vi "libssh2_channel_read_ex.vi"(8 "error in (no error)":errorcluster, 9 "buffer length":i32=1024, 10 "stream id":i32, 11 "channel":T1) -> (0 "error out":errorcluster, 2 "buffer":u8[](array[numeric]))   [LabVIEW 2017, in "libssh2.lvlib"]
doc: "Read data from a channel.\nAll channel streams have one standard input/output substream (<B>stream id</B> = 0), and may have up to 2^32 extended data streams as identified by the selected <B>stream id</B>. The SSH-2 protocol currently defines a standard stream ID of 1 to be the stderr substream."
uses:
  libssh2.lvlib
  Channel Refnum.ctl
  Acquire Session.vi
  Release Session.vi
  Not A Channel.vi
  <vilib>/Utility/error.llb/Error Cluster From Error Code.vi
  Global Settings.vi
  Read Channel Refnum.vi
  Read Session Refnum.vi
  <vilib>/Utility/semaphor.llb/Acquire Semaphore.vi
  <vilib>/Utility/semaphor.llb/Release Semaphore.vi
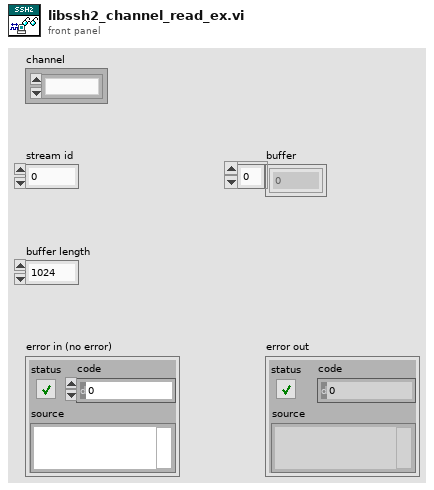
[diagram p1: front panel]
types:
  T1 = typedef "libssh2.lvlib/Channel Refnum.ctl" = refnum<k1>
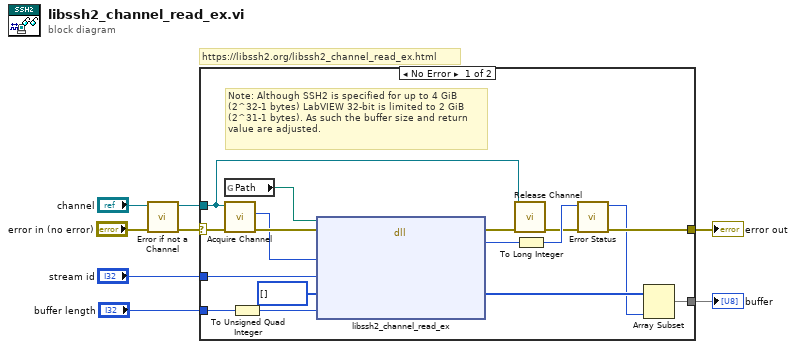
[diagram p0: block diagram]
diagram:
  # "https://libssh2.org/libssh2_channel_read_ex.html"
  n1 = call "Error if not a Channel.vi"("error in (no error)"="error in (no error)", "channel"="channel") -> ("error out"=w3:errorcluster, "channel out"=w1:T1)  [unwired: 8 in]
  n2 = case shown="No Error" w3 {
    selector: w3 -> [w22 w26]
    tunnel: "stream id" -> [w25 _]
    tunnel: "buffer length" -> [w24 _]
    tunnel: [w21 w26] -> w6
    tunnel: [w23 _] -> w5
    tunnel: w1 -> [w9 _]
    frame No Error {
      # "Note: Although SSH2 is specified for up to 4 GiB\n(2^32-1 bytes) LabVIEW 32-bit is limited to 2 GiB\n(2^31-1 bytes). As such the buffer size and return\nvalue are adjusted."
      n3 = global read "Global Settings.vi" "Path"() -> (w16:path)
      n4 = call "Acquire Channel.vi"("error in (no error)"=w22, "channel"=w9) -> ("error out"=w18:errorcluster, "LIBSSH2_CHANNEL*"=w17:u64)  [unwired: 8 in]
      n5 = To Unsigned Quad Integer(1:w24) -> (0:w12:u64)
      n6 = dll-call lib="?" fn="libssh2_channel_read_ex"(path in=w16, error in=w18, "channel"=w17, "stream_id"=w25, "buf"=u8[] [], "buflen"=w12) -> (error out=w20:errorcluster, "return value"=w15:i64, "buf"=w19:u8[])  [unwired: 4 in, 1 out]
      n7 = call "Release Channel.vi"("error in (no error)"=w20, "channel"=w9) -> ("error out"=w10:errorcluster)  [unwired: 9 in]
      n8 = To Long Integer(number=w15) -> (32bit integer=w14:i32)
      n9 = call "Error Status.vi"("error in (no error)"=w10, "return value"=w14) -> ("error out"=w21:errorcluster, "return value out"=w13:i32)  [unwired: 8 in]
      n10 = Array Subset(array=w19, length=w13) -> (w23:u8[])  [unwired: 1 in]
    }
    frame Error {
    }
  }
  "error out" <- w6
  "buffer" <- w5
